vi "Gserver_Query.vi"(8 "error in (no error)":errorcluster, 9 "Query":T1, 10 "Requester":string, 11 "FAMM in":refnum<class "FAMM.lvclass">) -> (0 "error out":errorcluster, 3 "FAMM out":refnum<class "FAMM.lvclass">)   [LabVIEW 2020, in "Sgraph_lib_V1.lvlib" / "FAMM.lvclass"]
doc: "Andre Koelewijn, 17 jan 2021\n\nThis VI will process a query as received from Gserver,\nthis query is a request for one of the Gviewer instances."
uses:
  FAMM.lvclass
  controls/FAMMrequest.ctl
  Gview/controls/Typedef_Live.ctl
  controls/FAMM_reply_datagram.ctl
  controls/FAMM_reply_WAQdata.ctl
  controls/FAMM_reply_EAQdata.ctl
  controls/FAMM_reply_PAQdata.ctl
  Gserver/controls/Typedef_QueryType.ctl
  FAMM.lvclass/FAMM.ctl
  DBAL/DBAL.lvclass
  PAQ-memory.lvclass
  Gview/Gviewer.lvclass
  Gserver/Gserver.lvclass
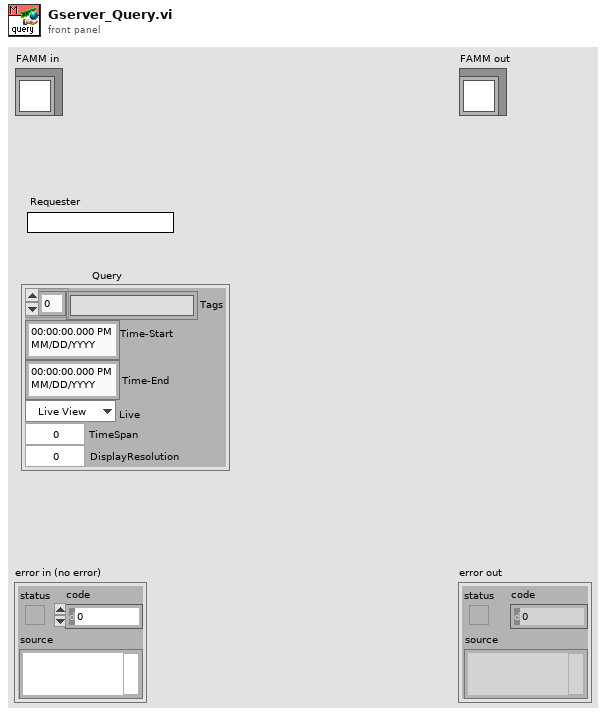
[diagram p1: front panel]
types:
  T1 = typedef "Sgraph_lib_V1.lvlib/FAMM.lvclass/FAMMrequest.ctl" = cluster{"Tags":string[], "Time-Start":timestamp, "Time-End":timestamp, "Live":T2, "TimeSpan":dbl, "DisplayResolution":i32}
  T2 = typedef "Sgraph_lib_V1.lvlib/Gviewer.lvclass/Typedef_Live.ctl" = enum16{"Live View", "Freeze"}
  T3 = typedef "Sgraph_lib_V1.lvlib/Gserver.lvclass/Typedef_QueryType.ctl" = enum16{"Subscribe", "DataRequest", "RequestAllTags", "RequestIniPath", "FAMMstarted", "SetClientOptions", "GviewerUpdate", "OpenNewGraph", "CloseClient", "CloseAllClients", "Close Gserver", "OpenMemoryMap", "MeMapDataRequest", "MeMapDataResponse"}
  T4 = typedef "Sgraph_lib_V1.lvlib/FAMM.lvclass/FAMM_reply_datagram.ctl" = cluster{"GraphName":string, "Time-Start":timestamp, "Time-End":timestamp, "TimeSpan":dbl, "Live":T2, "WAQ_section":T5, "EAQ_section":T6, "PAQ_section":T7, "Layer":i32}
  T5 = typedef "Sgraph_lib_V1.lvlib/FAMM.lvclass/FAMM_reply_WAQdata.ctl" = cluster{"Boolean":bool}
  T6 = typedef "Sgraph_lib_V1.lvlib/FAMM.lvclass/FAMM_reply_EAQdata.ctl" = cluster{"Boolean":bool}
  T7 = typedef "Sgraph_lib_V1.lvlib/FAMM.lvclass/FAMM_reply_PAQdata.ctl" = cluster{"Tags":string[], "time stamp":timestamp[], "DataSection":cluster{"data":dbl[], "max":dbl[], "min":dbl[], "Status":u32[]}[]}
  T8 = cluster{"time stamp":timestamp[], "DataSection":cluster{"data":dbl[], "max":dbl[], "min":dbl[], "Status":u32[]}[]}
  T9 = cluster{"data":dbl[], "max":dbl[], "min":dbl[], "Status":u32[]}[]
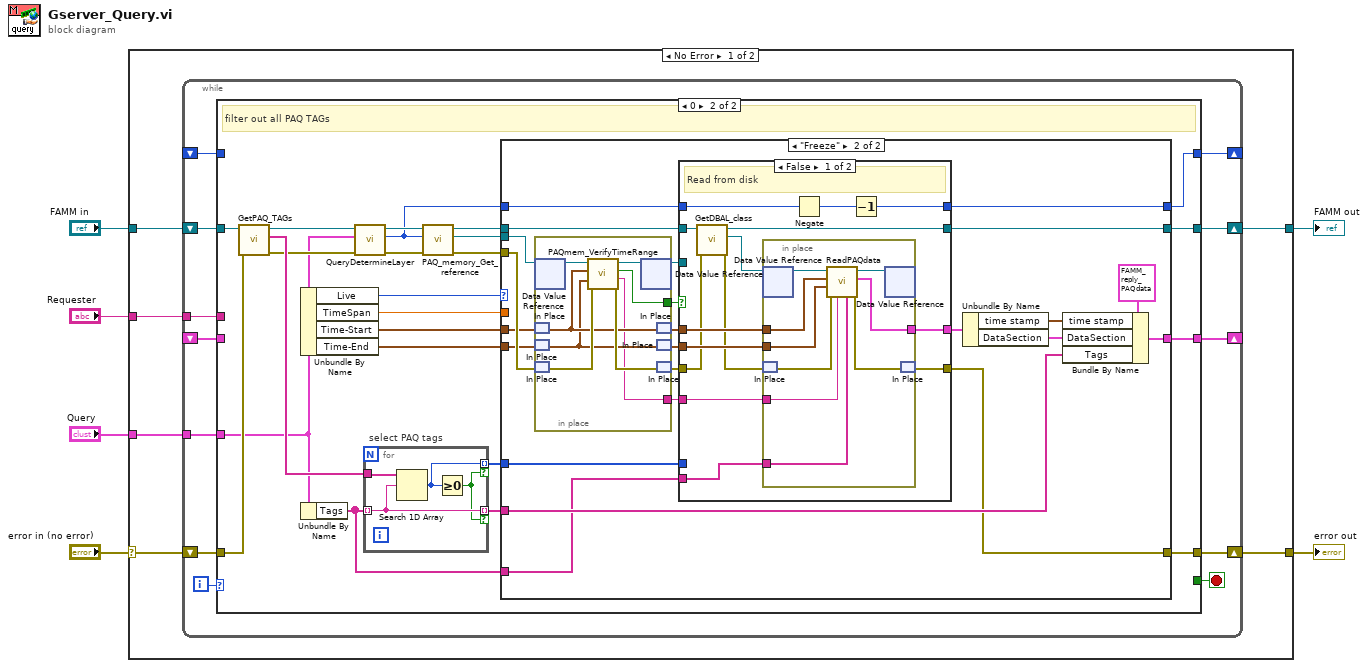
[diagram p0: block diagram]
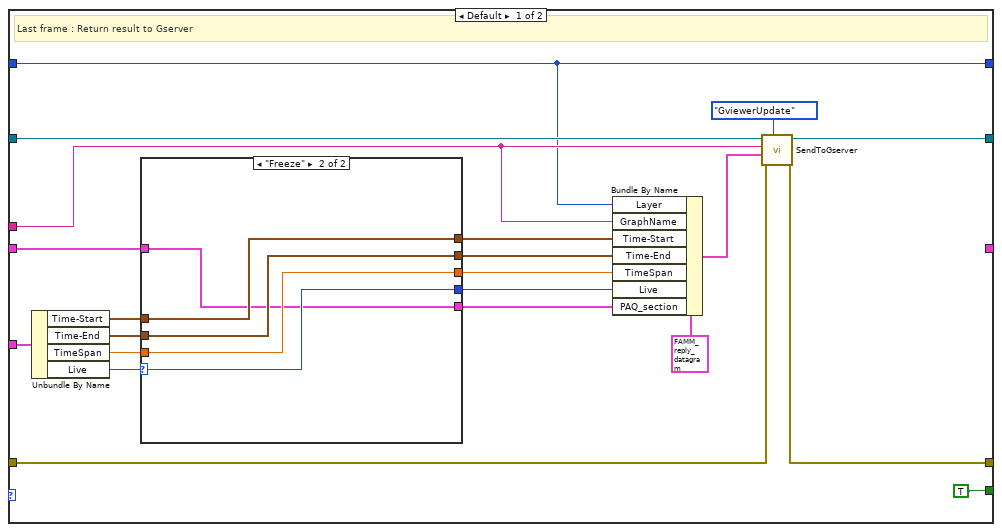
[diagram p2: hidden frame]
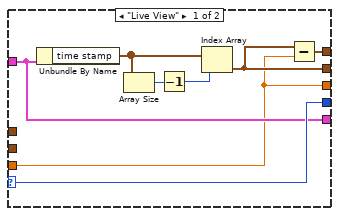
[diagram p3: hidden frame]
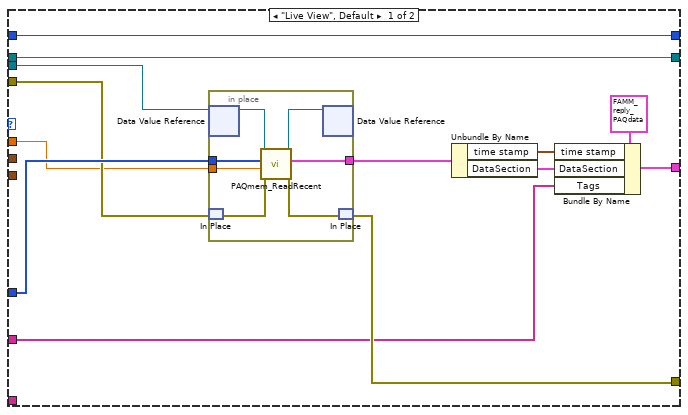
[diagram p4: hidden frame]
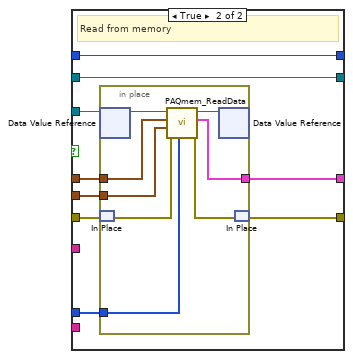
[diagram p5: hidden frame]
diagram:
  n1 = case shown="No Error" "error in (no error)" {
    selector: "error in (no error)" -> [w11 w178]
    tunnel: [w9 w178] -> w5
    tunnel: [w10 w177] -> w3
    tunnel: "FAMM in" -> [w12 w177]
    tunnel: "Requester" -> [w7 _]
    tunnel: "Query" -> [w8 _]
    frame No Error {
      n2 = while {
        shift-right: [w21] -> w10
        shift-left: w12 -> [w22]
        shift-right: [w19] -> w9
        shift-left: w11 -> [w20]
        tunnel: w8 -> [w18]
        shift-right: [w16] -> _
        shift-left: _ -> [w15]
        tunnel: w7 -> [w17]
        shift-right: [w14] -> _
        shift-left: _ -> [w13]
        i -> [w24]
        stop <- w23 stop-if-true
        n3 = case shown="0" w24 {
          tunnel: [TRUE _] -> w23
          tunnel: w22 -> [w43 w81]
          tunnel: [w44 w78] -> w21
          tunnel: w20 -> [w41 w79]
          tunnel: [w42 w77] -> w19
          tunnel: w18 -> [w38 w63]
          tunnel: [_ w62] -> w16
          tunnel: w15 -> [w28 _]
          tunnel: w17 -> [w40 _]
          tunnel: [w25 w59] -> w14
          tunnel: w13 -> [w25 _]
          frame Default {
            # "Last frame : Return result to Gserver"
            n4 = Unbundle By Name(w38) -> ("Time-Start"=w33:timestamp, "Time-End"=w31:timestamp, "TimeSpan"=w36:dbl, "Live"=w37:T2)
            n5 = case shown="\"Freeze\"" w37 {
              selector: w37 -> [w53 w58]
              tunnel: w36 -> [w47 w57]
              tunnel: [w47 w57] -> w35
              tunnel: [w53 w58] -> w34
              tunnel: w33 -> [_ w56]
              tunnel: [w46 w56] -> w32
              tunnel: w31 -> [_ w55]
              tunnel: [w48 w55] -> w30
              tunnel: w28 -> [w49 w54]
              tunnel: [w49 w54] -> w26
              frame "Live View" {
                n6 = Unbundle By Name(w49) -> ("time stamp"=w52:timestamp[])
                n7 = Array Size(array=w52) -> (size(s)=w51:i32)
                n8 = Decrement(x=w51) -> (x-1=w50:i32)
                n9 = Index Array(array=w52, index=w50) -> (element=w48:timestamp)
                n10 = Subtract(x=w48, y=w47) -> (x-y=w46:timestamp)
              }
              frame "Freeze" {
              }
            }
            n11 = Bundle By Name(cluster=T4 {"GraphName"="", "Time-Start"=timestamp(3693735326.5884657 s since 1904-01-01), "Time-End"=timestamp(3693738926.5884657 s since 1904-01-01), "TimeSpan"=3600.0, "Live"=enum."Live View", "WAQ_section"={"Boolean"=FALSE}, "EAQ_section"={"Boolean"=FALSE}, "PAQ_section"={"Tags"=[], "time stamp"=[timestamp(3693738906.0787926 s since 1904-01-01), timestamp(3693738907.07885 s since 1904-01-01), timestamp(3693738908.078907 s since 1904-01-01), timestamp(3693738909.0784645 s since 1904-01-01), timestamp(3693738910.078021 s since 1904-01-01), timestamp(3693738911.0780787 s since 1904-01-01), timestamp(3693738912.0781355 s since 1904-01-01), timestamp(3693738913.078193 s since 1904-01-01), timestamp(3693738914.07825 s since 1904-01-01), timestamp(3693738915.078307 s since 1904-01-01), timestamp(3693738916.0783644 s since 1904-01-01), timestamp(3693738917.0784216 s since 1904-01-01), timestamp(3693738918.078479 s since 1904-01-01), timestamp(3693738919.079036 s since 1904-01-01), timestamp(3693738920.0795937 s since 1904-01-01), timestamp(3693738921.079651 s since 1904-01-01), timestamp(3693738922.080208 s since 1904-01-01), timestamp(3693738923.080765 s since 1904-01-01), timestamp(3693738924.080822 s since 1904-01-01), timestamp(3693738925.080879 s since 1904-01-01), timestamp(3693738926.0809364 s since 1904-01-01)], "DataSection"=[{"data"=[0.025001418590545655, 0.025001442432403563, 0.025001442432403563, 0.024976420402526855, 0.025001418590545655, 0.025001442432403563, 0.025001418590545655, 0.025001442432403563, 0.025001418590545655, 0.02500143051147461, 0.02500143051147461, 0.02500143051147461, 0.025001418590545655, 0.025026440620422363, 0.025001442432403563, 0.025001418590545655, 0.025026440620422363, 0.025001418590545655, 0.025001442432403563, 0.025001418590545655, 0.025001442432403563], "max"=[0.025002002716064453, 0.025002002716064453, 0.027001380920410156, 0.025002002716064453, 0.025002002716064453, 0.025002002716064453, 0.025002002716064453, 0.025002002716064453, 0.025002002716064453, 0.025002002716064453, 0.025002002716064453, 0.025002002716064453, 0.025002002716064453, 0.026001453399658203, 0.025002002716064453, 0.025002002716064453, 0.026001930236816406, 0.025002002716064453, 0.025002002716064453, 0.025002002716064453, 0.025002002716064453], "min"=[0.025000572204589844, 0.025000572204589844, 0.023000717163085938, 0.024001598358154297, 0.025000572204589844, 0.025000572204589844, 0.025000572204589844, 0.025000572204589844, 0.025000572204589844, 0.025000572204589844, 0.025000572204589844, 0.025000572204589844, 0.025000572204589844, 0.025000572204589844, 0.025000572204589844, 0.025000572204589844, 0.025000572204589844, 0.025000572204589844, 0.025000572204589844, 0.025000572204589844, 0.025000572204589844], "Status"=[32, 32, 32, 32, 32, 32, 32, 32, 32, 32, 32, 32, 32, 32, 32, 32, 32, 32, 32, 32, 32]}, {"data"=[-0.9354747896064408, -0.8404284269564783, -0.7071607347032589, -0.5418428772577799, -0.35190732133675506, -0.14587999085598086, 0.0667803616892586, 0.2764042621476871, 0.4734603938185778, 0.6489887332802559, 0.7950082939099952, 0.9048796538456292, 0.9736070993342884, 0.9980611009504278, 0.9770997684259897, 0.9117044287198024, 0.804780917615083, 0.6612496881767144, 0.48770429821940564, 0.2919835550131608, 0.08298658586533915], "max"=[-0.8959308174823704, -0.7813847664948913, -0.6313098736866257, -0.45272075499094866, -0.2533811699487135, -0.04252038230785384, 0.1702734124585812, 0.3753254016660106, 0.563311520829305, 0.7256844818543676, 0.8550614257826367, 0.9455595807831805, 0.9930641768448534, 0.9999999409410515, 0.994868561200511, 0.9507995750699587, 0.8634987130737423, 0.736791128791916, 0.5766900244522951, 0.39036772701230454, 0.18629562188798668], "min"=[-0.9684220062635356, -0.8935455880916622, -0.7780405553946977, -0.6271589239650177, -0.44795195781971175, -0.24821082458062316, -0.03718357863555101, 0.17553401560557638, 0.38027060996619916, 0.5677163831595027, 0.7293489873127391, 0.8578186952327538, 0.9472843262210879, 0.993677989367111, 0.9524406630582044, 0.8661801494925992, 0.7403917173979886, 0.5810453180987437, 0.3952793148134019, 0.1915404908565982, -0.02090770788724533], "Status"=[32, 32, 32, 32, 32, 32, 32, 32, 32, 32, 32, 32, 32, 32, 32, 32, 32, 32, 32, 32, 32]}, {"data"=[216.71823637754036, 216.72123654939543, 216.72423687087658, 216.727235467406, 216.73023406403246, 216.73323423540242, 216.73623440725754, 216.73923457862756, 216.74223475041794, 216.74523492182033, 216.74823509364313, 216.75123526514253, 216.75423543673884, 216.75723665836912, 216.76023878024557, 216.76323895158325, 216.76624077346384, 216.76924229486355, 216.77224246675095, 216.77524263812097, 216.77824280984674], "max"=[216.71969896027196, 216.72269913316185, 216.72569930605175, 216.72869647671985, 216.73169664702274, 216.73469681991264, 216.73769699021554, 216.74069716310544, 216.7436973334083, 216.7466975050047, 216.7496976766011, 216.75269784819747, 216.75569801850037, 216.75870119102507, 216.76170136520844, 216.76470153551136, 216.76770470803604, 216.7707048783389, 216.7737050512288, 216.7767052215317, 216.7797053944216], "min"=[216.71677379377394, 216.71977396407684, 216.7227741382602, 216.7257743072696, 216.7287714818182, 216.7317716508276, 216.734771825011, 216.7377719953139, 216.7407721682038, 216.74377233850666, 216.74677251139656, 216.74977268169945, 216.75277285329582, 216.75577302489225, 216.7587761974169, 216.76177636771982, 216.7647765393162, 216.76777971054736, 216.77077988343726, 216.77378005374015, 216.77678022533655], "Status"=[32, 32, 32, 32, 32, 32, 32, 32, 32, 32, 32, 32, 32, 32, 32, 32, 32, 32, 32, 32, 32]}, {"data"=[0.0020000000000000005, 0.0020000000000000005, 0.0020000000000000005, 0.0020000000000000005, 0.0020000000000000005, 0.0020000000000000005, 0.0020000000000000005, 0.0020000000000000005, 0.0020000000000000005, 0.0020000000000000005, 0.0020000000000000005, 0.0020000000000000005, 0.0020000000000000005, 0.0020000000000000005, 0.0020000000000000005, 0.0020000000000000005, 0.0020000000000000005, 0.0020000000000000005, 0.0020000000000000005, 0.0020000000000000005, 0.0020000000000000005], "max"=[0.002, 0.002, 0.002, 0.002, 0.002, 0.002, 0.002, 0.002, 0.002, 0.002, 0.002, 0.002, 0.002, 0.002, 0.002, 0.002, 0.002, 0.002, 0.002, 0.002, 0.002], "min"=[0.002, 0.002, 0.002, 0.002, 0.002, 0.002, 0.002, 0.002, 0.002, 0.002, 0.002, 0.002, 0.002, 0.002, 0.002, 0.002, 0.002, 0.002, 0.002, 0.002, 0.002], "Status"=[32, 32, 32, 32, 32, 32, 32, 32, 32, 32, 32, 32, 32, 32, 32, 32, 32, 32, 32, 32, 32]}, {"data"=[-0.02066160993998472, -0.020661606639795653, -0.02066160333944171, -0.02066160004098581, -0.02066159674252958, -0.02066159344234105, -0.02066159014215198, -0.020661586841963318, -0.020661583541774515, -0.020661580241585716, -0.020661576941396715, -0.020661573641208048, -0.020661570341019446, -0.020661567039675467, -0.02066156373734151, -0.02066156043715298, -0.020661557135149104, -0.02066155383347565, -0.020661550533286516, -0.020661547233097717, -0.020661543932908776], "max"=[-0.020661608331142632, -0.02066160503095477, -0.020661601730764232, -0.0206615984338765, -0.020661595133688627, -0.020661591833498097, -0.020661588533310234, -0.020661585233119697, -0.02066158193293183, -0.02066157863274396, -0.0206615753325561, -0.020661572032365558, -0.020661568732180363, -0.02066156542868969, -0.02066156212849916, -0.02066155882831129, -0.020661555524820626, -0.020661552224632763, -0.020661548924444894, -0.020661545624257028, -0.02066154232406649], "min"=[-0.020661611548827206, -0.020661608248639336, -0.020661604948448806, -0.020661601648260933, -0.020661598351370537, -0.020661595051182664, -0.020661591750992133, -0.02066158845080694, -0.020661585150616397, -0.020661581850428535, -0.020661578550237997, -0.020661575250050135, -0.020661571949862262, -0.02066156864967173, -0.020661565346183727, -0.020661562045995865, -0.020661558745805334, -0.02066155544231733, -0.0206615521421268, -0.02066154884193893, -0.020661545541751064], "Status"=[32, 32, 32, 32, 32, 32, 32, 32, 32, 32, 32, 32, 32, 32, 32, 32, 32, 32, 32, 32, 32]}]}, "Layer"=0} ("GviewerUpdate"), "Layer"=w25, "GraphName"=w40, "Time-Start"=w32, "Time-End"=w30, "TimeSpan"=w35, "Live"=w34, "PAQ_section"=w26) -> (w39:T4)
            n12 = call "SendToGserver.vi"("Query_type"=Typedef_QueryType."GviewerUpdate", "error in (no error)"=w41, "data"=w39, "Address"=w40, "FAMM in"=w43) -> ("error out"=w42:errorcluster, "FAMM out"=w44:refnum<class "FAMM.lvclass">)  [unwired: 5 in]
          }
          frame 0 {
            # "filter out all PAQ TAGs"
            n13 = call "GetPAQ_TAGs.vi"("error in (no error)"=w79, "FAMM in"=w81) -> ("error out"=w67:errorcluster, "PAQ_TAGs"=w80:string[], "FAMM out"=w65:refnum<class "FAMM.lvclass">)  [unwired: 7 in]
            n14 = Unbundle By Name(w63) -> ("Live"=w76:T2, "TimeSpan"=w70:dbl, "Time-Start"=w69:timestamp, "Time-End"=w68:timestamp)
            n15 = Unbundle By Name(w63) -> ("Tags"=w61:string[])
            n16 = call "QueryDetermineLayer.vi"("error in (no error)"=w67, "Query"=w63, "FAMM in"=w65) -> ("error out"=w66:errorcluster, "Memory_Layer"=w60:i32, "FAMM out"=w64:refnum<class "FAMM.lvclass">)  [unwired: 6 in]
            n17 = for "select PAQ tags" {
              tunnel: w61 -> [w175] mode=indexing
              tunnel: w80 -> [w176]
              tunnel: [w175] -> w75 mode=indexing if=w173
              tunnel: [w174] -> w71 mode=indexing if=w173
              n18 = Search 1D Array(1D array=w176, element=w175) -> (index of element=w174:i32)  [unwired: 1 in]
              n19 = Greater Or Equal To 0?(x=w174) -> (x >= 0?=w173:bool)
            }
            n20 = call "PAQ_memory_Get_reference.vi"("error in (no error)"=w66, "PAQ_Layer"=w60, "FAMM in"=w64) -> ("error out"=w73:errorcluster, "PAQ_memory"=w72:refnum<data-value>, "FAMM out"=w74:refnum<class "FAMM.lvclass">)  [unwired: 6 in]
            n21 = case shown="\"Freeze\"" w76 {
              tunnel: w74 -> [w89 w106]
              tunnel: w73 -> [w91 w124]
              tunnel: [w89 w112] -> w78
              tunnel: [w92 w113] -> w77
              tunnel: w75 -> [w85 w119]
              tunnel: w72 -> [w94 w123]
              tunnel: w71 -> [w93 w111]
              tunnel: w70 -> [w90 _]
              tunnel: [w84 w118] -> w62
              tunnel: w69 -> [_ w117]
              tunnel: w68 -> [_ w116]
              tunnel: w61 -> [_ w104]
              tunnel: w60 -> [w82 w103]
              tunnel: [w82 w102] -> w59
              frame "Live View", Default {
                n22 = in-place {
                  in-place-border: w93 -> [w97]
                  in-place-border: w90 -> [w96]
                  in-place-border: [w95] -> w88
                  n23 = in-place-dvr #1(w94) -> (w101:refnum<class "PAQ-memory.lvclass">)  [unwired: 1 out]
                  n24 = in-place-match #2(w91) -> (w99:errorcluster)
                  n25 = call "PAQmem_ReadRecent.vi"("error in (no error)"=w99, "TimeSpan(sec)"=w96, "TagsIndices"=w97, "PAQ-memory in"=w101) -> ("error out"=w98:errorcluster, "PAQ_section"=w95:T8, "PAQ-memory out"=w100:refnum<class "PAQ-memory.lvclass">)  [unwired: 5 in]
                  n26 = in-place-dvr #1(w100) -> ()  [unwired: 2 out]
                  n27 = in-place-match #2(w98) -> (w92:errorcluster)
                }
                n28 = Unbundle By Name(w88) -> ("time stamp"=w87:timestamp[], "DataSection"=w86:T9)
                n29 = Bundle By Name(cluster=T7 {"Tags"=[], "time stamp"=[timestamp(3693738906.0787926 s since 1904-01-01), timestamp(3693738907.07885 s since 1904-01-01), timestamp(3693738908.078907 s since 1904-01-01), timestamp(3693738909.0784645 s since 1904-01-01), timestamp(3693738910.078021 s since 1904-01-01), timestamp(3693738911.0780787 s since 1904-01-01), timestamp(3693738912.0781355 s since 1904-01-01), timestamp(3693738913.078193 s since 1904-01-01), timestamp(3693738914.07825 s since 1904-01-01), timestamp(3693738915.078307 s since 1904-01-01), timestamp(3693738916.0783644 s since 1904-01-01), timestamp(3693738917.0784216 s since 1904-01-01), timestamp(3693738918.078479 s since 1904-01-01), timestamp(3693738919.079036 s since 1904-01-01), timestamp(3693738920.0795937 s since 1904-01-01), timestamp(3693738921.079651 s since 1904-01-01), timestamp(3693738922.080208 s since 1904-01-01), timestamp(3693738923.080765 s since 1904-01-01), timestamp(3693738924.080822 s since 1904-01-01), timestamp(3693738925.080879 s since 1904-01-01), timestamp(3693738926.0809364 s since 1904-01-01)], "DataSection"=[{"data"=[0.025001418590545655, 0.025001442432403563, 0.025001442432403563, 0.024976420402526855, 0.025001418590545655, 0.025001442432403563, 0.025001418590545655, 0.025001442432403563, 0.025001418590545655, 0.02500143051147461, 0.02500143051147461, 0.02500143051147461, 0.025001418590545655, 0.025026440620422363, 0.025001442432403563, 0.025001418590545655, 0.025026440620422363, 0.025001418590545655, 0.025001442432403563, 0.025001418590545655, 0.025001442432403563], "max"=[0.025002002716064453, 0.025002002716064453, 0.027001380920410156, 0.025002002716064453, 0.025002002716064453, 0.025002002716064453, 0.025002002716064453, 0.025002002716064453, 0.025002002716064453, 0.025002002716064453, 0.025002002716064453, 0.025002002716064453, 0.025002002716064453, 0.026001453399658203, 0.025002002716064453, 0.025002002716064453, 0.026001930236816406, 0.025002002716064453, 0.025002002716064453, 0.025002002716064453, 0.025002002716064453], "min"=[0.025000572204589844, 0.025000572204589844, 0.023000717163085938, 0.024001598358154297, 0.025000572204589844, 0.025000572204589844, 0.025000572204589844, 0.025000572204589844, 0.025000572204589844, 0.025000572204589844, 0.025000572204589844, 0.025000572204589844, 0.025000572204589844, 0.025000572204589844, 0.025000572204589844, 0.025000572204589844, 0.025000572204589844, 0.025000572204589844, 0.025000572204589844, 0.025000572204589844, 0.025000572204589844], "Status"=[32, 32, 32, 32, 32, 32, 32, 32, 32, 32, 32, 32, 32, 32, 32, 32, 32, 32, 32, 32, 32]}, {"data"=[-0.9354747896064408, -0.8404284269564783, -0.7071607347032589, -0.5418428772577799, -0.35190732133675506, -0.14587999085598086, 0.0667803616892586, 0.2764042621476871, 0.4734603938185778, 0.6489887332802559, 0.7950082939099952, 0.9048796538456292, 0.9736070993342884, 0.9980611009504278, 0.9770997684259897, 0.9117044287198024, 0.804780917615083, 0.6612496881767144, 0.48770429821940564, 0.2919835550131608, 0.08298658586533915], "max"=[-0.8959308174823704, -0.7813847664948913, -0.6313098736866257, -0.45272075499094866, -0.2533811699487135, -0.04252038230785384, 0.1702734124585812, 0.3753254016660106, 0.563311520829305, 0.7256844818543676, 0.8550614257826367, 0.9455595807831805, 0.9930641768448534, 0.9999999409410515, 0.994868561200511, 0.9507995750699587, 0.8634987130737423, 0.736791128791916, 0.5766900244522951, 0.39036772701230454, 0.18629562188798668], "min"=[-0.9684220062635356, -0.8935455880916622, -0.7780405553946977, -0.6271589239650177, -0.44795195781971175, -0.24821082458062316, -0.03718357863555101, 0.17553401560557638, 0.38027060996619916, 0.5677163831595027, 0.7293489873127391, 0.8578186952327538, 0.9472843262210879, 0.993677989367111, 0.9524406630582044, 0.8661801494925992, 0.7403917173979886, 0.5810453180987437, 0.3952793148134019, 0.1915404908565982, -0.02090770788724533], "Status"=[32, 32, 32, 32, 32, 32, 32, 32, 32, 32, 32, 32, 32, 32, 32, 32, 32, 32, 32, 32, 32]}, {"data"=[216.71823637754036, 216.72123654939543, 216.72423687087658, 216.727235467406, 216.73023406403246, 216.73323423540242, 216.73623440725754, 216.73923457862756, 216.74223475041794, 216.74523492182033, 216.74823509364313, 216.75123526514253, 216.75423543673884, 216.75723665836912, 216.76023878024557, 216.76323895158325, 216.76624077346384, 216.76924229486355, 216.77224246675095, 216.77524263812097, 216.77824280984674], "max"=[216.71969896027196, 216.72269913316185, 216.72569930605175, 216.72869647671985, 216.73169664702274, 216.73469681991264, 216.73769699021554, 216.74069716310544, 216.7436973334083, 216.7466975050047, 216.7496976766011, 216.75269784819747, 216.75569801850037, 216.75870119102507, 216.76170136520844, 216.76470153551136, 216.76770470803604, 216.7707048783389, 216.7737050512288, 216.7767052215317, 216.7797053944216], "min"=[216.71677379377394, 216.71977396407684, 216.7227741382602, 216.7257743072696, 216.7287714818182, 216.7317716508276, 216.734771825011, 216.7377719953139, 216.7407721682038, 216.74377233850666, 216.74677251139656, 216.74977268169945, 216.75277285329582, 216.75577302489225, 216.7587761974169, 216.76177636771982, 216.7647765393162, 216.76777971054736, 216.77077988343726, 216.77378005374015, 216.77678022533655], "Status"=[32, 32, 32, 32, 32, 32, 32, 32, 32, 32, 32, 32, 32, 32, 32, 32, 32, 32, 32, 32, 32]}, {"data"=[0.0020000000000000005, 0.0020000000000000005, 0.0020000000000000005, 0.0020000000000000005, 0.0020000000000000005, 0.0020000000000000005, 0.0020000000000000005, 0.0020000000000000005, 0.0020000000000000005, 0.0020000000000000005, 0.0020000000000000005, 0.0020000000000000005, 0.0020000000000000005, 0.0020000000000000005, 0.0020000000000000005, 0.0020000000000000005, 0.0020000000000000005, 0.0020000000000000005, 0.0020000000000000005, 0.0020000000000000005, 0.0020000000000000005], "max"=[0.002, 0.002, 0.002, 0.002, 0.002, 0.002, 0.002, 0.002, 0.002, 0.002, 0.002, 0.002, 0.002, 0.002, 0.002, 0.002, 0.002, 0.002, 0.002, 0.002, 0.002], "min"=[0.002, 0.002, 0.002, 0.002, 0.002, 0.002, 0.002, 0.002, 0.002, 0.002, 0.002, 0.002, 0.002, 0.002, 0.002, 0.002, 0.002, 0.002, 0.002, 0.002, 0.002], "Status"=[32, 32, 32, 32, 32, 32, 32, 32, 32, 32, 32, 32, 32, 32, 32, 32, 32, 32, 32, 32, 32]}, {"data"=[-0.02066160993998472, -0.020661606639795653, -0.02066160333944171, -0.02066160004098581, -0.02066159674252958, -0.02066159344234105, -0.02066159014215198, -0.020661586841963318, -0.020661583541774515, -0.020661580241585716, -0.020661576941396715, -0.020661573641208048, -0.020661570341019446, -0.020661567039675467, -0.02066156373734151, -0.02066156043715298, -0.020661557135149104, -0.02066155383347565, -0.020661550533286516, -0.020661547233097717, -0.020661543932908776], "max"=[-0.020661608331142632, -0.02066160503095477, -0.020661601730764232, -0.0206615984338765, -0.020661595133688627, -0.020661591833498097, -0.020661588533310234, -0.020661585233119697, -0.02066158193293183, -0.02066157863274396, -0.0206615753325561, -0.020661572032365558, -0.020661568732180363, -0.02066156542868969, -0.02066156212849916, -0.02066155882831129, -0.020661555524820626, -0.020661552224632763, -0.020661548924444894, -0.020661545624257028, -0.02066154232406649], "min"=[-0.020661611548827206, -0.020661608248639336, -0.020661604948448806, -0.020661601648260933, -0.020661598351370537, -0.020661595051182664, -0.020661591750992133, -0.02066158845080694, -0.020661585150616397, -0.020661581850428535, -0.020661578550237997, -0.020661575250050135, -0.020661571949862262, -0.02066156864967173, -0.020661565346183727, -0.020661562045995865, -0.020661558745805334, -0.02066155544231733, -0.0206615521421268, -0.02066154884193893, -0.020661545541751064], "Status"=[32, 32, 32, 32, 32, 32, 32, 32, 32, 32, 32, 32, 32, 32, 32, 32, 32, 32, 32, 32, 32]}]} ("PAQ_section"), "time stamp"=w87, "DataSection"=w86, "Tags"=w85) -> (w84:T7)
              }
              frame "Freeze" {
                n30 = in-place {
                  in-place-border: [w168] -> w115
                  in-place-border: [w165] -> w105
                  n31 = in-place-dvr #3(w123) -> (w172:refnum<class "PAQ-memory.lvclass">)  [unwired: 1 out]
                  n32 = in-place-match #4(w117) -> (w167:timestamp)
                  n33 = in-place-match #5(w116) -> (w166:timestamp)
                  n34 = in-place-match #6(w124) -> (w170:errorcluster)
                  n35 = call "PAQmem_VerifyTimeRange.vi"("error in (no error)"=w170, "Time-End"=w166, "Time-Start"=w167, "PAQ-memory in"=w172) -> ("error out"=w169:errorcluster, "TableName"=w165:string, "All data in memory range"=w168:bool, "PAQ-memory out"=w171:refnum<class "PAQ-memory.lvclass">)  [unwired: 4 in]
                  n36 = in-place-dvr #3(w171) -> (w108:refnum<data-value>)  [unwired: 1 out]
                  n37 = in-place-match #4(w167) -> (w110:timestamp)
                  n38 = in-place-match #5(w166) -> (w109:timestamp)
                  n39 = in-place-match #6(w169) -> (w114:errorcluster)
                }
                n40 = case shown="False" w115 {
                  tunnel: w114 -> [w131 w155]
                  tunnel: [w135 w154] -> w113
                  tunnel: w106 -> [w137 w156]
                  tunnel: [w138 w156] -> w112
                  tunnel: w111 -> [_ w150]
                  tunnel: w110 -> [w134 w152]
                  tunnel: w109 -> [w133 w151]
                  tunnel: w108 -> [_ w153]
                  tunnel: [w130 w149] -> w107
                  tunnel: w105 -> [w129 _]
                  tunnel: w104 -> [w128 _]
                  tunnel: w103 -> [w127 w148]
                  tunnel: [w125 w148] -> w102
                  frame False {
                    # "Read from disk"
                    n41 = call "GetDBAL_class.vi"("error in (no error)"=w131, "FAMM in"=w137) -> ("error out"=w132:errorcluster, "DBAL_class"=w136:refnum<data-value>, "FAMM out"=w138:refnum<class "FAMM.lvclass">)  [unwired: 7 in]
                    n42 = in-place {
                      in-place-border: w134 -> [w146]
                      in-place-border: w133 -> [w145]
                      in-place-border: w128 -> [w139]
                      in-place-border: [w141] -> w130
                      in-place-border: w129 -> [w140]
                      n43 = in-place-dvr #7(w136) -> (w147:refnum<class "DBAL.lvclass">)  [unwired: 1 out]
                      n44 = in-place-match #8(w132) -> (w144:errorcluster)
                      n45 = call-dynamic "ReadPAQdata.vi"("Tags"=w139, "TableName"=w140, "error in (no error)"=w144, "Time-End"=w145, "Time-Start"=w146, "DBAL in"=w147) -> ("error out"=w143:errorcluster, "PAQ_section"=w141:T8, "DBAL out"=w142:refnum<class "DBAL.lvclass">)  [unwired: 3 in]
                      n46 = in-place-dvr #7(w142) -> ()  [unwired: 2 out]
                      n47 = in-place-match #8(w143) -> (w135:errorcluster)
                    }
                    n48 = Negate(x=w127) -> (-x=w126:i32)
                    n49 = Decrement(x=w126) -> (x-1=w125:i32)
                  }
                  frame True {
                    # "Read from memory"
                    n50 = in-place {
                      in-place-border: w152 -> [w160]
                      in-place-border: w151 -> [w159]
                      in-place-border: w150 -> [w157]
                      in-place-border: [w158] -> w149
                      n51 = in-place-dvr #9(w153) -> (w164:refnum<class "PAQ-memory.lvclass">)  [unwired: 1 out]
                      n52 = in-place-match #10(w155) -> (w161:errorcluster)
                      n53 = call "PAQmem_ReadData.vi"("TagsIndices"=w157, "error in (no error)"=w161, "Time-End"=w159, "Time-Start"=w160, "PAQ-memory in"=w164) -> ("error out"=w162:errorcluster, "PAQ_section"=w158:T8, "PAQ-memory out"=w163:refnum<class "PAQ-memory.lvclass">)  [unwired: 4 in]
                      n54 = in-place-dvr #9(w163) -> ()  [unwired: 2 out]
                      n55 = in-place-match #10(w162) -> (w154:errorcluster)
                    }
                  }
                }
                n56 = Unbundle By Name(w107) -> ("time stamp"=w122:timestamp[], "DataSection"=w121:T9)
                n57 = Bundle By Name(cluster=T7 {"Tags"=[], "time stamp"=[timestamp(3693738906.0787926 s since 1904-01-01), timestamp(3693738907.07885 s since 1904-01-01), timestamp(3693738908.078907 s since 1904-01-01), timestamp(3693738909.0784645 s since 1904-01-01), timestamp(3693738910.078021 s since 1904-01-01), timestamp(3693738911.0780787 s since 1904-01-01), timestamp(3693738912.0781355 s since 1904-01-01), timestamp(3693738913.078193 s since 1904-01-01), timestamp(3693738914.07825 s since 1904-01-01), timestamp(3693738915.078307 s since 1904-01-01), timestamp(3693738916.0783644 s since 1904-01-01), timestamp(3693738917.0784216 s since 1904-01-01), timestamp(3693738918.078479 s since 1904-01-01), timestamp(3693738919.079036 s since 1904-01-01), timestamp(3693738920.0795937 s since 1904-01-01), timestamp(3693738921.079651 s since 1904-01-01), timestamp(3693738922.080208 s since 1904-01-01), timestamp(3693738923.080765 s since 1904-01-01), timestamp(3693738924.080822 s since 1904-01-01), timestamp(3693738925.080879 s since 1904-01-01), timestamp(3693738926.0809364 s since 1904-01-01)], "DataSection"=[{"data"=[0.025001418590545655, 0.025001442432403563, 0.025001442432403563, 0.024976420402526855, 0.025001418590545655, 0.025001442432403563, 0.025001418590545655, 0.025001442432403563, 0.025001418590545655, 0.02500143051147461, 0.02500143051147461, 0.02500143051147461, 0.025001418590545655, 0.025026440620422363, 0.025001442432403563, 0.025001418590545655, 0.025026440620422363, 0.025001418590545655, 0.025001442432403563, 0.025001418590545655, 0.025001442432403563], "max"=[0.025002002716064453, 0.025002002716064453, 0.027001380920410156, 0.025002002716064453, 0.025002002716064453, 0.025002002716064453, 0.025002002716064453, 0.025002002716064453, 0.025002002716064453, 0.025002002716064453, 0.025002002716064453, 0.025002002716064453, 0.025002002716064453, 0.026001453399658203, 0.025002002716064453, 0.025002002716064453, 0.026001930236816406, 0.025002002716064453, 0.025002002716064453, 0.025002002716064453, 0.025002002716064453], "min"=[0.025000572204589844, 0.025000572204589844, 0.023000717163085938, 0.024001598358154297, 0.025000572204589844, 0.025000572204589844, 0.025000572204589844, 0.025000572204589844, 0.025000572204589844, 0.025000572204589844, 0.025000572204589844, 0.025000572204589844, 0.025000572204589844, 0.025000572204589844, 0.025000572204589844, 0.025000572204589844, 0.025000572204589844, 0.025000572204589844, 0.025000572204589844, 0.025000572204589844, 0.025000572204589844], "Status"=[32, 32, 32, 32, 32, 32, 32, 32, 32, 32, 32, 32, 32, 32, 32, 32, 32, 32, 32, 32, 32]}, {"data"=[-0.9354747896064408, -0.8404284269564783, -0.7071607347032589, -0.5418428772577799, -0.35190732133675506, -0.14587999085598086, 0.0667803616892586, 0.2764042621476871, 0.4734603938185778, 0.6489887332802559, 0.7950082939099952, 0.9048796538456292, 0.9736070993342884, 0.9980611009504278, 0.9770997684259897, 0.9117044287198024, 0.804780917615083, 0.6612496881767144, 0.48770429821940564, 0.2919835550131608, 0.08298658586533915], "max"=[-0.8959308174823704, -0.7813847664948913, -0.6313098736866257, -0.45272075499094866, -0.2533811699487135, -0.04252038230785384, 0.1702734124585812, 0.3753254016660106, 0.563311520829305, 0.7256844818543676, 0.8550614257826367, 0.9455595807831805, 0.9930641768448534, 0.9999999409410515, 0.994868561200511, 0.9507995750699587, 0.8634987130737423, 0.736791128791916, 0.5766900244522951, 0.39036772701230454, 0.18629562188798668], "min"=[-0.9684220062635356, -0.8935455880916622, -0.7780405553946977, -0.6271589239650177, -0.44795195781971175, -0.24821082458062316, -0.03718357863555101, 0.17553401560557638, 0.38027060996619916, 0.5677163831595027, 0.7293489873127391, 0.8578186952327538, 0.9472843262210879, 0.993677989367111, 0.9524406630582044, 0.8661801494925992, 0.7403917173979886, 0.5810453180987437, 0.3952793148134019, 0.1915404908565982, -0.02090770788724533], "Status"=[32, 32, 32, 32, 32, 32, 32, 32, 32, 32, 32, 32, 32, 32, 32, 32, 32, 32, 32, 32, 32]}, {"data"=[216.71823637754036, 216.72123654939543, 216.72423687087658, 216.727235467406, 216.73023406403246, 216.73323423540242, 216.73623440725754, 216.73923457862756, 216.74223475041794, 216.74523492182033, 216.74823509364313, 216.75123526514253, 216.75423543673884, 216.75723665836912, 216.76023878024557, 216.76323895158325, 216.76624077346384, 216.76924229486355, 216.77224246675095, 216.77524263812097, 216.77824280984674], "max"=[216.71969896027196, 216.72269913316185, 216.72569930605175, 216.72869647671985, 216.73169664702274, 216.73469681991264, 216.73769699021554, 216.74069716310544, 216.7436973334083, 216.7466975050047, 216.7496976766011, 216.75269784819747, 216.75569801850037, 216.75870119102507, 216.76170136520844, 216.76470153551136, 216.76770470803604, 216.7707048783389, 216.7737050512288, 216.7767052215317, 216.7797053944216], "min"=[216.71677379377394, 216.71977396407684, 216.7227741382602, 216.7257743072696, 216.7287714818182, 216.7317716508276, 216.734771825011, 216.7377719953139, 216.7407721682038, 216.74377233850666, 216.74677251139656, 216.74977268169945, 216.75277285329582, 216.75577302489225, 216.7587761974169, 216.76177636771982, 216.7647765393162, 216.76777971054736, 216.77077988343726, 216.77378005374015, 216.77678022533655], "Status"=[32, 32, 32, 32, 32, 32, 32, 32, 32, 32, 32, 32, 32, 32, 32, 32, 32, 32, 32, 32, 32]}, {"data"=[0.0020000000000000005, 0.0020000000000000005, 0.0020000000000000005, 0.0020000000000000005, 0.0020000000000000005, 0.0020000000000000005, 0.0020000000000000005, 0.0020000000000000005, 0.0020000000000000005, 0.0020000000000000005, 0.0020000000000000005, 0.0020000000000000005, 0.0020000000000000005, 0.0020000000000000005, 0.0020000000000000005, 0.0020000000000000005, 0.0020000000000000005, 0.0020000000000000005, 0.0020000000000000005, 0.0020000000000000005, 0.0020000000000000005], "max"=[0.002, 0.002, 0.002, 0.002, 0.002, 0.002, 0.002, 0.002, 0.002, 0.002, 0.002, 0.002, 0.002, 0.002, 0.002, 0.002, 0.002, 0.002, 0.002, 0.002, 0.002], "min"=[0.002, 0.002, 0.002, 0.002, 0.002, 0.002, 0.002, 0.002, 0.002, 0.002, 0.002, 0.002, 0.002, 0.002, 0.002, 0.002, 0.002, 0.002, 0.002, 0.002, 0.002], "Status"=[32, 32, 32, 32, 32, 32, 32, 32, 32, 32, 32, 32, 32, 32, 32, 32, 32, 32, 32, 32, 32]}, {"data"=[-0.02066160993998472, -0.020661606639795653, -0.02066160333944171, -0.02066160004098581, -0.02066159674252958, -0.02066159344234105, -0.02066159014215198, -0.020661586841963318, -0.020661583541774515, -0.020661580241585716, -0.020661576941396715, -0.020661573641208048, -0.020661570341019446, -0.020661567039675467, -0.02066156373734151, -0.02066156043715298, -0.020661557135149104, -0.02066155383347565, -0.020661550533286516, -0.020661547233097717, -0.020661543932908776], "max"=[-0.020661608331142632, -0.02066160503095477, -0.020661601730764232, -0.0206615984338765, -0.020661595133688627, -0.020661591833498097, -0.020661588533310234, -0.020661585233119697, -0.02066158193293183, -0.02066157863274396, -0.0206615753325561, -0.020661572032365558, -0.020661568732180363, -0.02066156542868969, -0.02066156212849916, -0.02066155882831129, -0.020661555524820626, -0.020661552224632763, -0.020661548924444894, -0.020661545624257028, -0.02066154232406649], "min"=[-0.020661611548827206, -0.020661608248639336, -0.020661604948448806, -0.020661601648260933, -0.020661598351370537, -0.020661595051182664, -0.020661591750992133, -0.02066158845080694, -0.020661585150616397, -0.020661581850428535, -0.020661578550237997, -0.020661575250050135, -0.020661571949862262, -0.02066156864967173, -0.020661565346183727, -0.020661562045995865, -0.020661558745805334, -0.02066155544231733, -0.0206615521421268, -0.02066154884193893, -0.020661545541751064], "Status"=[32, 32, 32, 32, 32, 32, 32, 32, 32, 32, 32, 32, 32, 32, 32, 32, 32, 32, 32, 32, 32]}]} ("PAQ_section"), "time stamp"=w122, "DataSection"=w121, "Tags"=w119) -> (w118:T7)
              }
            }
          }
        }
      }
    }
    frame Error {
    }
  }
  "error out" <- w5
  "FAMM out" <- w3
